vi "Read VISA resource name.vi"(8 "error in (no error)":errorcluster, 11 "CO3000 in":refnum<class "CO3000.lvclass">) -> (0 "error out":errorcluster, 2 "VISA resource name":refnum<visa-resource-name>, 3 "CO3000 out":refnum<class "CO3000.lvclass">)   [LabVIEW 2023, in "Turn Table and Mast.lvlib" / "CO3000.lvclass"]
uses:
  CO3000.lvclass
  CO3000.lvclass/CO3000.ctl
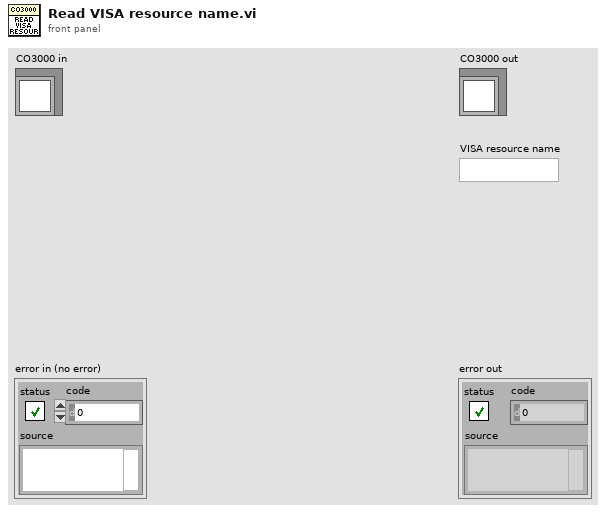
[diagram p1: front panel]
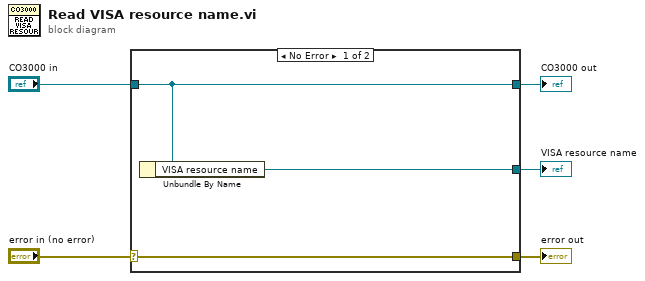
[diagram p0: block diagram]
diagram:
  n1 = case shown="No Error" "error in (no error)" {
    selector: "error in (no error)" -> [w8 w9]
    tunnel: [w8 w9] -> w4
    tunnel: [w7 w10] -> w2
    tunnel: "CO3000 in" -> [w7 w10]
    tunnel: [w6 _] -> w1
    frame No Error {
      n2 = Unbundle By Name(w7) -> ("VISA resource name"=w6:refnum<visa-resource-name>)
    }
    frame Error {
    }
  }
  "error out" <- w4
  "CO3000 out" <- w2
  "VISA resource name" <- w1
